vi "Add OutputOffset to Waveform.vi"(8 "error in (no error)":errorcluster, 10 "WFM in":waveform(dbl)[](array[waveform]), 11 "Instrument.DAQ":refnum<class "Instrument.DAQ.lvclass">) -> (0 "error out":errorcluster, 2 "WFM out":waveform(dbl)[](array[waveform]), 3 "Instrument.DAQ out":refnum<class "Instrument.DAQ.lvclass">)   [LabVIEW 2019, in "Instrument.Lockin.lvlib" / "Instrument.DAQ.lvclass"]
uses:
  Instrument.DAQ.lvclass
  Instrument.DAQ.lvclass/Instrument.DAQ.ctl
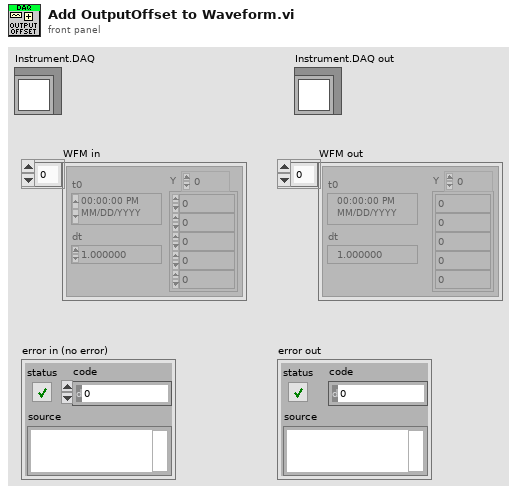
[diagram p1: front panel]
types:
  T1 = typedef "Instrument.Lockin.lvlib/Instrument.DAQ.lvclass/Channel.Offset--Cluster--Array.ctl" = T2[]
  T2 = typedef "Instrument.Lockin.lvlib/Instrument.DAQ.lvclass/Channel.Offset--Cluster.ctl" = cluster{"Channel":string, "Offset":dbl}
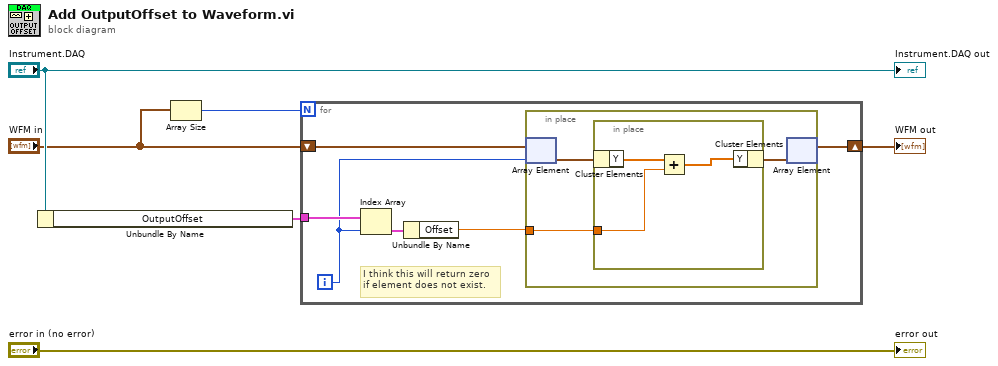
[diagram p0: block diagram]
diagram:
  n1 = Unbundle By Name("Instrument.DAQ") -> ("OutputOffset"=w1:T1)
  n2 = Array Size(array="WFM in") -> (size(s)=w2:i32)
  n3 = for {
    N: w2 -> [_]
    tunnel: w1 -> [w10]
    shift-right: [w12] -> w6
    shift-left: "WFM in" -> [w11]
    i -> [w9]
    # "I think this will return zero\nif element does not exist."
    n4 = Index Array(array=w10, index=w9) -> (element=w8:T2)
    n5 = Unbundle By Name(w8) -> ("Offset"=w7:dbl)
    n6 = in-place {
      in-place-border: w7 -> [w13]
      n7 = in-place-array #1(w11, w9) -> (w15:waveform(dbl))
      n8 = in-place {
        in-place-border: w13 -> [w17]
        n9 = in-place-cluster #2(w15) -> ("Y"=w18:dbl[])
        n10 = Add(x=w18, y=w17) -> (x+y=w16:dbl[])
        n11 = in-place-cluster #2("Y"=w16) -> (w14:waveform(dbl))
      }
      n12 = in-place-array #1(w14) -> (w12:waveform(dbl)[])  [unwired: 1 out]
    }
  }
  "WFM out" <- w6
  "error out" <- "error in (no error)"
  "Instrument.DAQ out" <- "Instrument.DAQ"
